vi "send_requests.vi"(8 "error in":errorcluster, 9 "Python env version":string="3.12", 10 "Path to client.py":path, 11 "Python env directory":path) -> (0 "error out":errorcluster)   [LabVIEW 2023]
uses:
  <vilib>/Python/Open Venv Python Session.vi
panel:
  out "scaled array":dbl[](array[numeric])
  in  "array":dbl[](array[numeric])=[1.0, 2.0]
  in  "scaling factor":dbl=2.0
  out "services available":string[](array[string])
  in  "Service name (Python or LabVIEW)":string="Python"
  in  "y (add)":dbl=2.0 format="%#_13g"
  in  "x (add)":dbl=1.0 format="%#_13g"
  in  "string to reverse":string="Hello, world!"
  out "reversed string":string
  out "addition result":dbl
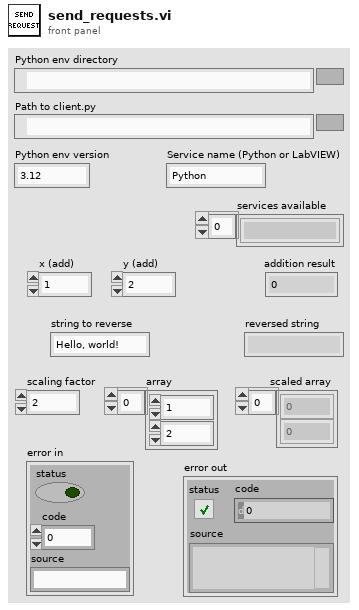
[diagram p1: front panel]
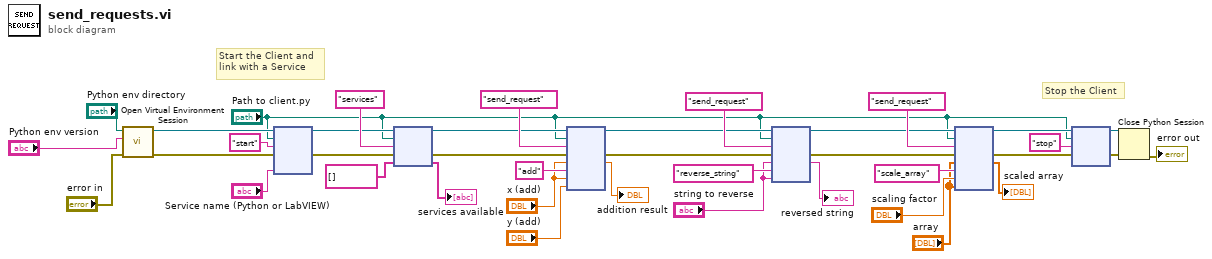
[diagram p0: block diagram]
diagram:
  # "Stop the Client"
  # "Start the Client and link with a Service"
  n1 = call-poly <vilib>:"Open Virtual Environment Session.vi"("error in (no error)"="error in", "Python version"="Python env version", "Env path"="Python env directory") -> ("error out"=w36:errorcluster, "session out"=w37:refnum<k35>)  [unwired: 7 in]
  n2 = node(w37, "Path to client.py", "start" ("function name"), w36, "Service name (Python or LabVIEW)") -> (w13:refnum<k35>, w14:errorcluster)  [unwired: 3 in, 2 out]
  n3 = node(w13, "Path to client.py", "services" ("function name"), w14, string[] [] ("return type")) -> (w12:refnum<k35>, w11:errorcluster, →"services available":string[])  [unwired: 2 out]
  n4 = node(w12, "Path to client.py", "send_request" ("function name"), w11, "x (add)", "add" ("parameter"), "x (add)", "y (add)") -> (w18:refnum<k35>, w21:errorcluster, →"addition result":dbl)  [unwired: 3 in, 2 out]
  n5 = node(w18, "Path to client.py", "send_request" ("function name"), w21, "string to reverse", "reverse_string" ("parameter"), "string to reverse") -> (w6:refnum<k35>, w7:errorcluster, →"reversed string":string)  [unwired: 2 in, 2 out]
  n6 = node(w6, "Path to client.py", "send_request" ("function name"), w7, "array", "scale_array" ("parameter"), "scaling factor", "array") -> (w5:refnum<k35>, w3:errorcluster, →"scaled array":dbl[])  [unwired: 3 in, 2 out]
  n7 = node(w5, "Path to client.py", "stop" ("function name"), w3) -> (w33:refnum<k35>, w30:errorcluster)  [unwired: 2 in, 2 out]
  n8 = Close Python Session(session in=w33, error in=w30) -> (11:→"error out":errorcluster)
